vi "ASD Color Label.vi"(8 "Level Composition":string[](array[string]), 11 "Color":u32[](array[numeric])) -> (3 "Label":T1)   [LabVIEW 2018]
panel:
  out "7":u32(colorbox)
  out "6":u32(colorbox)
  out "5":u32(colorbox)
  out "4":u32(colorbox)
  out "3":u32(colorbox)
  out "2":u32(colorbox)
  out "1":u32(colorbox)
  out "0":u32(colorbox)
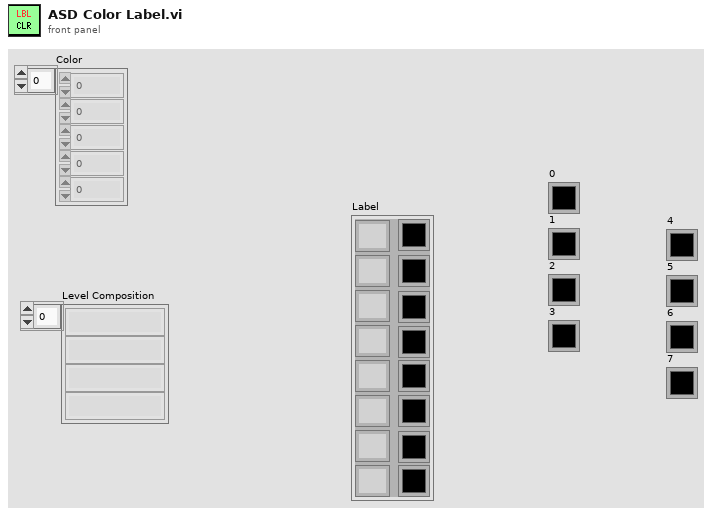
[diagram p1: front panel]
types:
  T1 = cluster{"カラーボックス":u32, "カラーボックス 4":u32, "カラーボックス 2":u32, "カラーボックス 5":u32, "カラーボックス 3":u32, "カラーボックス 6":u32, "カラーボックス 7":u32, "カラーボックス 8":u32, "B0":string, "B1":string, "B2":string, "B3":string, "B4":string, "B5":string, "B6":string, "B7":string}
  T2 = cluster{"Base Color":u32, "Base Color":u32, "Base Color":u32, "Base Color":u32, "Base Color":u32, "Base Color":u32, "Base Color":u32, "Base Color":u32, "Base Charactor":string, "Base Charactor":string, "Base Charactor":string, "Base Charactor":string, "Base Charactor":string, "Base Charactor":string, "Base Charactor":string, "Base Charactor":string}
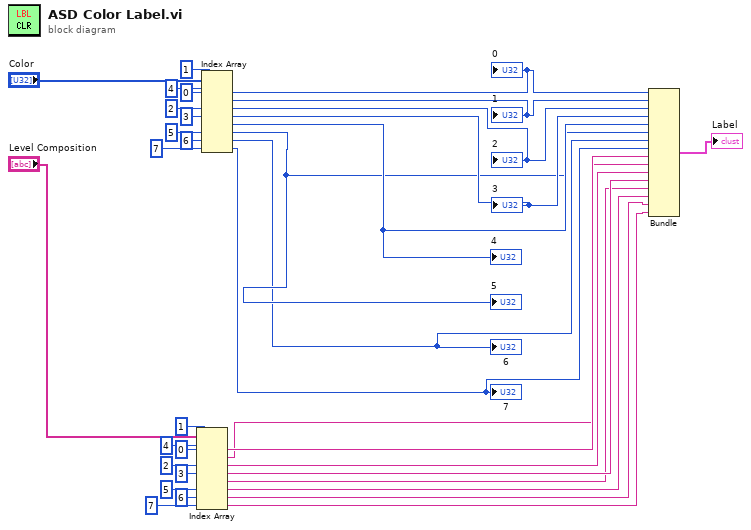
[diagram p0: block diagram]
diagram:
  n1 = Index Array(array="Level Composition", index #1=0 ("指標"), index #2=1 ("指標"), index #3=2 ("指標"), index #4=3 ("指標"), index #5=4 ("指標"), index #6=5 ("指標"), index #7=6 ("指標"), index #8=7 ("指標")) -> (element #1=w9:string, element #2=w8:string, element #3=w6:string, element #4=w5:string, element #5=w4:string, element #6=w3:string, element #7=w2:string, element #8=w1:string)
  n2 = Index Array(array="Color", index #1=0 ("指標"), index #2=1 ("指標"), index #3=2 ("指標"), index #4=3 ("指標"), index #5=4 ("指標"), index #6=5 ("指標"), index #7=6 ("指標"), index #8=7 ("指標")) -> (element #1=w27:u32, element #2=w26:u32, element #3=w25:u32, element #4=w24:u32, element #5=w23:u32, element #6=w22:u32, element #7=w21:u32, element #8=w20:u32)
  "0" <- w27
  "1" <- w26
  "2" <- w25
  "3" <- w24
  "4" <- w23
  "5" <- w22
  "6" <- w21
  "7" <- w20
  n3 = Bundle("Base Color"=w27, "Base Color"=w26, "Base Color"=w25, "Base Color"=w24, "Base Color"=w23, "Base Color"=w22, "Base Color"=w21, "Base Color"=w20, "Base Charactor"=w9, "Base Charactor"=w8, "Base Charactor"=w6, "Base Charactor"=w5, "Base Charactor"=w4, "Base Charactor"=w3, "Base Charactor"=w2, "Base Charactor"=w1) -> (→"Label":T2)  [unwired: 1 in]
